vi "MQTT QoS - Expect Reception.vi"(0 "MQTT Reference":T2, 5 "Packet ID":u16, 7 "Message":u8[](array[numeric]), 9 "MessageType":T1=enum."PUBREC", 11 "Error In":errorcluster) -> (4 "MQTT Reference":T2, 8 "Duplicate?":bool, 15 "Error Out":errorcluster)   [LabVIEW 2019, in "KoRE-MQTT.lvlib"]
doc: "Copyright (c) 2025 KoRElibs.com\nSPDX-License-Identifier: EUPL-1.2\n\nThis VI is licensed under the European Union Public License (EUPL) Version 1.2. You may use this VI unmodified in proprietary works. If you distribute a modified version of this file, the modified file must be released under the EUPL-1.2. Full license: https://joinup.ec.europa.eu/asset/eupl/eupl/1.2/"
uses:
  KoRE-MQTT.lvlib
  Public/TypeDefs/MQTT Client Session.ctl
  TypeDefs/MQTT Packet - Type.ctl
  TypeDefs/MQTT Client Session - Data Value Reference.ctl
  Public/TypeDefs/MQTT Client Session - Data.ctl
  Public/TypeDefs/MQTT Property - Will.ctl
  Public/TypeDefs/MQTT Property - CONNECT.ctl
  TypeDefs/MQTT Subscription - Info.ctl
  TypeDefs/MQTT QoS - In-flight Data.ctl
panel:
  out "DEBUG":variant
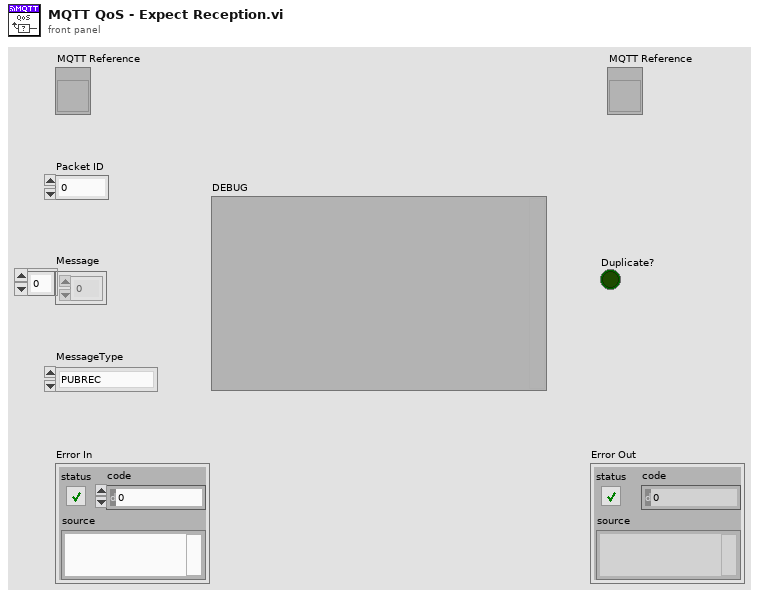
[diagram p1: front panel]
types:
  T1 = typedef "KoRE-MQTT.lvlib/MQTT Packet - Type.ctl" = enum32{"Reserved", "CONNECT", "CONNACK", "PUBLISH", "PUBACK", "PUBREC", "PUBREL", "PUBCOMP", "SUBSCRIBE", "SUBACK", "UNSUBSCRIBE", "UNSUBACK", "PINGREQ", "PINGRESP", "DISCONNECT", "AUTH"}
  T2 = typedef "KoRE-MQTT.lvlib/MQTT Client Session.ctl" = refnum<vi>
  T3 = typedef "KoRE-MQTT.lvlib/MQTT QoS - In-flight Data.ctl" = cluster{"Time":u32, "Message":u8[]}
  T4 = typedef "KoRE-MQTT.lvlib/MQTT Client Session - Data Value Reference.ctl" = refnum<data-value>
  T5 = typedef "KoRE-MQTT.lvlib/MQTT Client Session - Data.ctl" = cluster{"TCP ref":refnum<k5>, "Next Packet Id":u16, "Version":u8, "Host":string, "Port":u16, "Ping Delta":u32, "Username":string, "Password":string, "Will QoS":u8, "Will Retain":bool, "Will Topic":string, "Will Payload":string, "TCP Timeout":i32, "Semaphore":T6, "In-Flight Messages":variant, "Close":bool, "Last Send":u32, "Keep Alive":u16, "Last Ping RTT":u32, "Last Ping":u32, "Will Properties":T7[], "Session Expiry Interval":u32, "Maximum QoS":u8, "Retain Available":bool, "Server Maximum Packet Size":u32, "Client Identifier":string, "Server Topic Alias Maximum":u16, "Wildcard Subscription Available":bool, "Subscription Identifier Available":bool, "Shared Subscription Available":bool, "Connect Properties":T8[], "Client Maximum Packet Size":u32, "Client Topic Alias Maximum":u16, "Server Receive Maximum":u16, "Client Receive Maximum":u16, "TLS cfg":refnum<k36>, "Subscriptions":T9[]}
  T6 = typedef "Semaphore RefNum" = refnum<k1>
  T7 = typedef "KoRE-MQTT.lvlib/MQTT Property - Will.ctl" = cluster{"Property":u8, "Value":string}
  T8 = typedef "KoRE-MQTT.lvlib/MQTT Property - CONNECT.ctl" = cluster{"Property":u8, "Value":string}
  T9 = typedef "KoRE-MQTT.lvlib/MQTT Subscription - Info.ctl" = cluster{"Packet Id":u16, "Index":u16, "Identifier":u32, "QoS":u8, "Topic Filter":string, "Reason Code":u8, "Reason String":string, "Granted":bool}
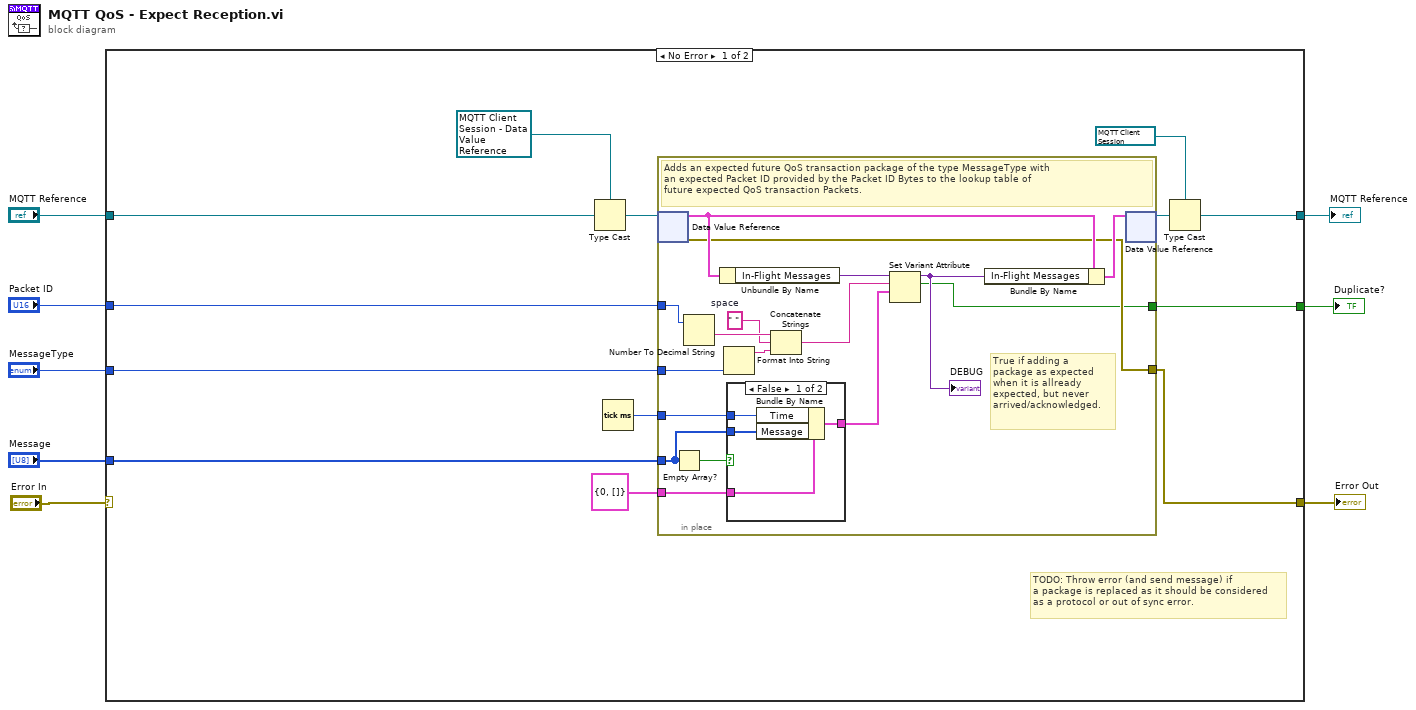
[diagram p0: block diagram]
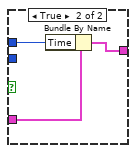
[diagram p2: hidden frame]
diagram:
  n1 = case shown="No Error" "Error In" {
    selector: "Error In" -> [_ w46]
    tunnel: "MQTT Reference" -> [w21 w47]
    tunnel: [w16 w47] -> w7
    tunnel: "Packet ID" -> [w15 _]
    tunnel: "MessageType" -> [w14 _]
    tunnel: [w13 w46] -> w4
    tunnel: [w12 _] -> w2
    tunnel: "Message" -> [w10 _]
    frame No Error {
      # "TODO: Throw error (and send message) if\na package is replaced as it should be considered\nas a protocol or out of sync error."
      n2 = Type Cast(type=T4 refnum ("data value reference"), x=w21) -> (*(type *) &x=w20:T4)
      n3 = Tick Count (ms)() -> (millisecond timer value=w9:u32)
      n4 = in-place {
        in-place-border: w15 -> [w27]
        in-place-border: w14 -> [w34]
        in-place-border: [w30] -> w13
        in-place-border: [w29] -> w12
        in-place-border: T3 {"Time"=0, "Message"=[]} -> [w26]
        in-place-border: w10 -> [w22]
        in-place-border: w9 -> [w24]
        w28 = " "  # space
        # "True if adding a\npackage as expected\nwhen it is allready\nexpected, but never\narrived/acknowledged."
        # "Adds an expected future QoS transaction package of the type MessageType with \nan expected Packet ID provided by the Packet ID Bytes to the lookup table of \nfuture expected QoS transaction Packets."
        n5 = in-place-dvr #1(w20) -> (w37:T5, w30:errorcluster)
        n6 = Empty Array?(array=w22) -> (empty?=w23:bool)
        n7 = Number To Decimal String(number=w27) -> (decimal integer string=w32:string)  [unwired: 1 in]
        n8 = Unbundle By Name(w37) -> ("In-Flight Messages"=w36:variant)
        n9 = Format Into String(w34) -> (resulting string=w33:string)  [unwired: 3 in, 1 out]
        n10 = case shown="False" w23 {
          tunnel: w26 -> [w40 w45]
          tunnel: [w41 w44] -> w25
          tunnel: w24 -> [w42 w43]
          tunnel: w22 -> [w39 _]
          frame False {
            n11 = Bundle By Name(cluster=w40, "Time"=w42, "Message"=w39) -> (w41:T3)
          }
          frame True {
            n12 = Bundle By Name(cluster=w45, "Time"=w43) -> (w44:T3)
          }
        }
        n13 = Concatenate Strings(w32, w28, w33) -> (w31:string)
        n14 = Set Variant Attribute(Variant=w36, name=w31, value=w25) -> (Variant out=w35:variant, replaced=w29:bool)  [unwired: 1 in, 1 out]
        "DEBUG" <- w35
        n15 = Bundle By Name(cluster=w37, "In-Flight Messages"=w35) -> (w38:T5)
        n16 = in-place-dvr #1(w38) -> (w18:T4)  [unwired: 1 out]
      }
      n17 = Type Cast(type=T2 refnum ("mqtt ref"), x=w18) -> (*(type *) &x=w16:T2)
    }
    frame Error {
    }
  }
  "MQTT Reference" <- w7
  "Error Out" <- w4
  "Duplicate?" <- w2
